vi "Edit Row.vi"   [LabVIEW 2013, in "DataGrid.lvlib" / "DataTable.lvclass"]
uses:
  DataTable.lvclass
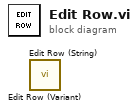
[diagram p0: block diagram]
diagram:
  n1 = call "Edit Row (Variant).vi"() -> ()  [unwired: 10 in, 2 out]
  n2 = call "Edit Row (String).vi"() -> ()  [unwired: 10 in, 2 out]
